vi "ZM-HWM-close.vi"(8 "error in (no error)":errorcluster, 11 "ZM-HWM-hardware_manager in":refnum<class "ZM-HWM-hardware_manager.lvclass">) -> (0 "error out":errorcluster, 3 "ZM-HWM-hardware_manager out":refnum<class "ZM-HWM-hardware_manager.lvclass">)   [LabVIEW 2020, in "ZM-HWM-hardware_manager.lvlib" / "ZM-HWM-hardware_manager.lvclass"]
doc: "Destroys the hardware manager's stop user event, called at the end of Actor Core and after a failed create. Release errors (an event never created) are ignored; error in passes through."
uses:
  ZM-HWM-hardware_manager.lvclass
  ZM-HWM-hardware_manager.lvclass/ZM-HWM-hardware_manager.ctl
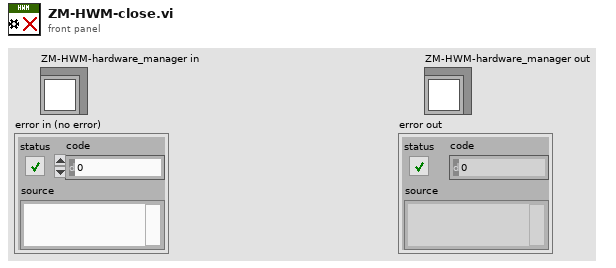
[diagram p1: front panel]
types:
  T1 = typedef "ZM-HWM-hardware_manager.lvlib/ZM-HWM-hardware_manager.lvclass/ZM-HWM-EVENTS.ctl" = cluster{"stop":refnum<user-event>}
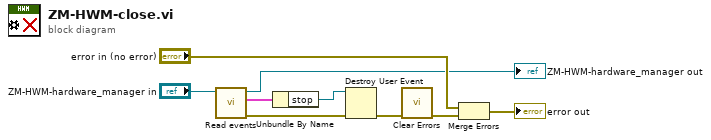
[diagram p0: block diagram]
diagram:
  n1 = call "Read events.vi"("ZM-HWM-hardware_manager in"="ZM-HWM-hardware_manager in") -> ("error out"=w6:errorcluster, "ZM-HWM-EVENTS"=w8:T1, "ZM-HWM-hardware_manager out"=→"ZM-HWM-hardware_manager out":refnum<class "ZM-HWM-hardware_manager.lvclass">)  [unwired: 8 in]
  n2 = Unbundle By Name(w8) -> ("stop"=w7:refnum<user-event>)
  n3 = Destroy User Event(user event=w7, error in=w6) -> (error out=w5:errorcluster)
  n4 = call <vilib>:"Clear Errors.vi"("error in (no error)"=w5) -> ("error out"=w3:errorcluster)  [unwired: 5 in, 1 out]
  n5 = Merge Errors("error in (no error)", w3) -> (→"error out":errorcluster)
